vi "Merge Limelight Data.vi"() -> ()   [LabVIEW 2025]
uses:
  <vilib>/Rock Robotics/WPI/DriverStation/WPI_DriverStationRobotMode2.ctl
  <vilib>/Rock Robotics/Network Tables/NT Read Numeric Array.vi
  <vilib>/Rock Robotics/Network Tables/NT Read Number.vi
  <vilib>/Rock Robotics/Network Tables/NT Write Numeric Array.vi
  Framework/Robot Global Data.vi
  <vilib>/Rock Robotics/Network Tables/NT Write String.vi
panel:
  out "What Camera are we seeing out of?":i32
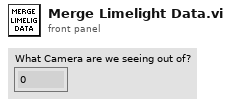
[diagram p1: front panel]
types:
  T1 = typedef "WPI_DriverStationRobotMode2.ctl" = enum16{"Autonomous Disabled", "Autonomous Enabled", "Teleop Disabled", "Teleop Enabled", "Disconnected", "Finish", "Test Disabled", "Test Enabled", "Emergency Stopped"}
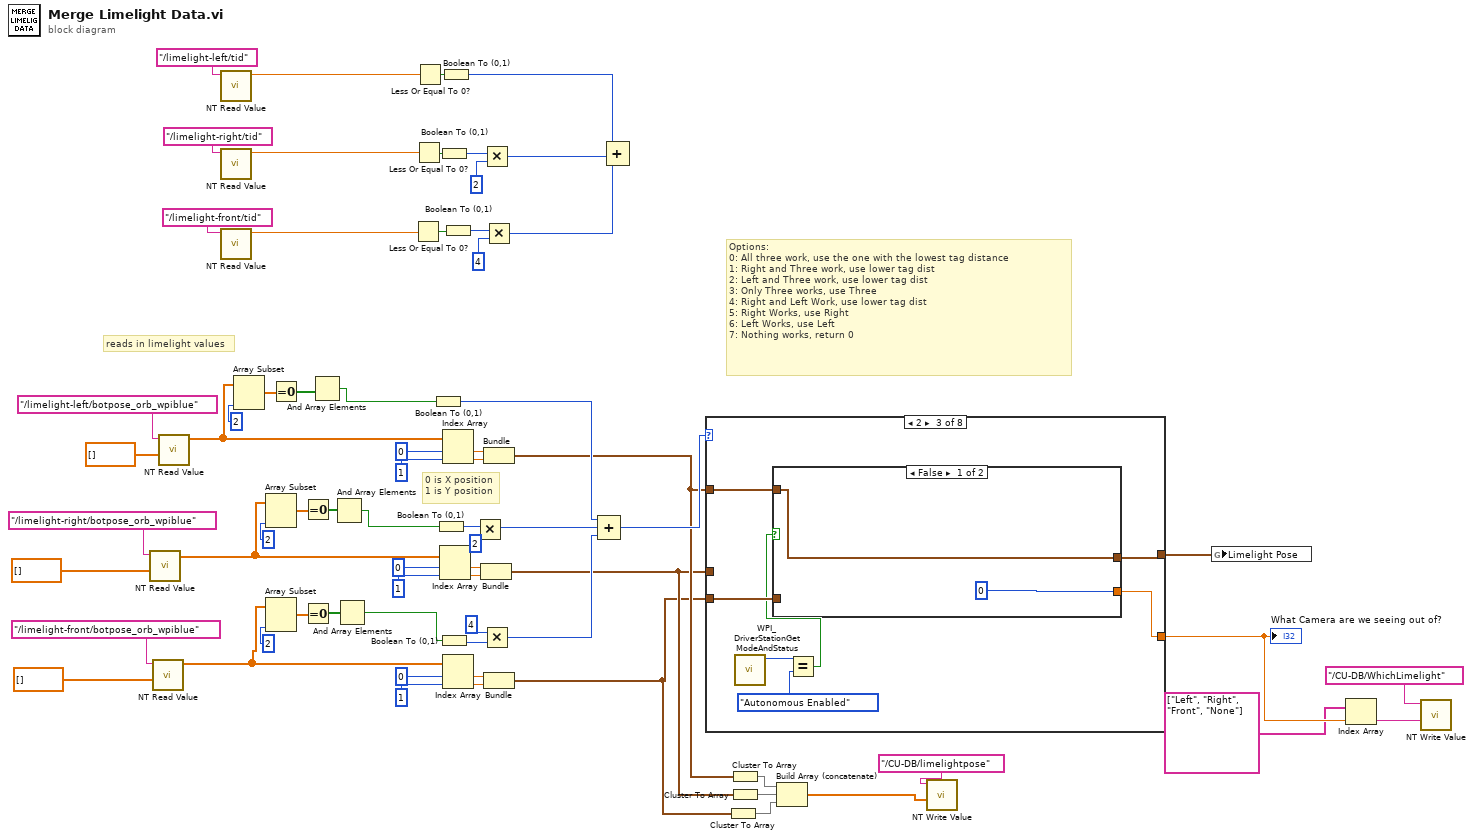
[diagram p0: block diagram]
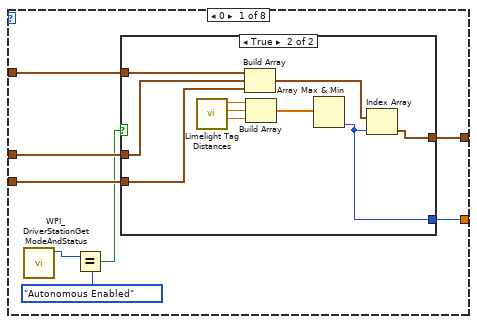
[diagram p2: hidden frame]
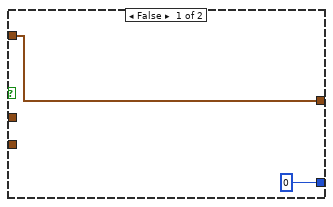
[diagram p3: hidden frame]
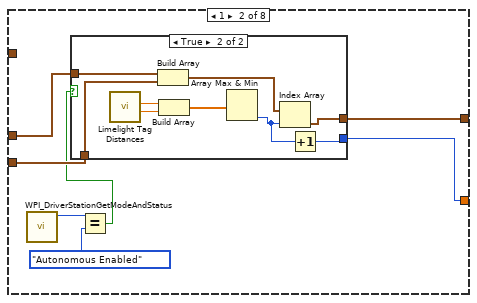
[diagram p4: hidden frame]
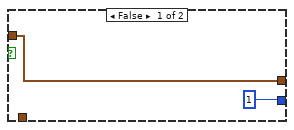
[diagram p5: hidden frame]
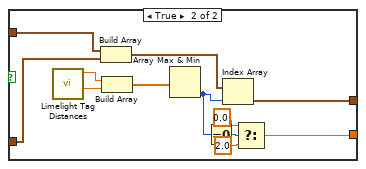
[diagram p6: hidden frame]
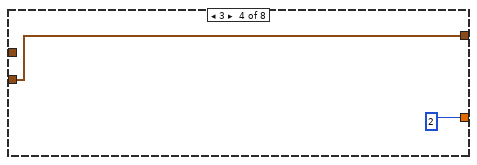
[diagram p7: hidden frame]
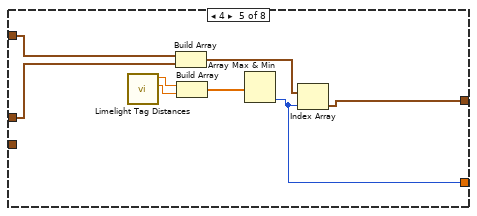
[diagram p8: hidden frame]
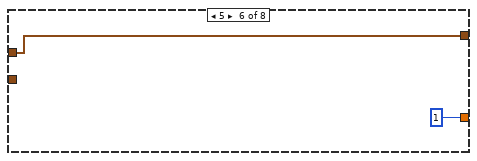
[diagram p9: hidden frame]
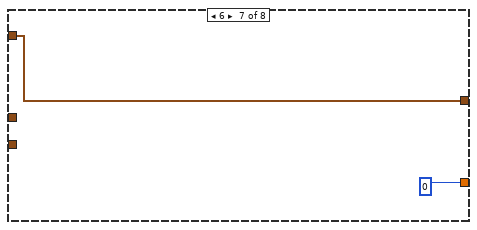
[diagram p10: hidden frame]
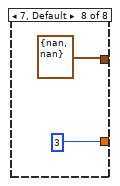
[diagram p11: hidden frame]
diagram:
  # "Options:\n0: All three work, use the one with the lowest tag distance\n1: Right and Three work, use lower tag dist\n2: Left and Three work, use lower tag dist\n3: Only Three works, use Three\n4: Right and Left Work, use lower tag dist\n5: Right Works, use Right\n6: Left Works, use Left\n7: Nothing works, return 0"
  # "reads in limelight values"
  # "0 is X position\n1 is Y position"
  n1 = call-poly <vilib>:"NT Read Value.vi"("default value"=dbl[] [], "name"="/limelight-right/botpose_orb_wpiblue") -> ("value"=w22:dbl[])  [unwired: 7 in, 2 out]
  n2 = call-poly <vilib>:"NT Read Value.vi"("default value"=dbl[] [], "name"="/limelight-front/botpose_orb_wpiblue") -> ("value"=w19:dbl[])  [unwired: 7 in, 2 out]
  n3 = call-poly <vilib>:"NT Read Value.vi"("default value"=dbl[] [], "name"="/limelight-left/botpose_orb_wpiblue") -> ("value"=w27:dbl[])  [unwired: 7 in, 2 out]
  n4 = call-poly <vilib>:"NT Read Value.vi"("name"="/limelight-left/tid") -> ("value"=w45:dbl)  [unwired: 8 in, 2 out]
  n5 = call-poly <vilib>:"NT Read Value.vi"("name"="/limelight-right/tid") -> ("value"=w44:dbl)  [unwired: 8 in, 2 out]
  n6 = call-poly <vilib>:"NT Read Value.vi"("name"="/limelight-front/tid") -> ("value"=w43:dbl)  [unwired: 8 in, 2 out]
  n7 = Array Subset(array=w27, length=2) -> (w25:dbl[])  [unwired: 1 in]
  n8 = Array Subset(array=w22, length=2) -> (w23:dbl[])  [unwired: 1 in]
  n9 = Array Subset(array=w19, length=2) -> (w20:dbl[])  [unwired: 1 in]
  n10 = Equal To 0?(x=w25) -> (x = 0?=w13:bool[])
  n11 = Equal To 0?(x=w23) -> (x = 0?=w15:bool[])
  n12 = Equal To 0?(x=w20) -> (x = 0?=w17:bool[])
  n13 = And Array Elements(Boolean array=w13) -> (logical AND=w12:bool)
  n14 = And Array Elements(Boolean array=w15) -> (logical AND=w14:bool)
  n15 = And Array Elements(Boolean array=w17) -> (logical AND=w16:bool)
  n16 = Less Or Equal To 0?(x=w43) -> (x <= 0?=w42:bool)
  n17 = Less Or Equal To 0?(x=w44) -> (x <= 0?=w41:bool)
  n18 = Less Or Equal To 0?(x=w45) -> (x <= 0?=w40:bool)
  n19 = Boolean To (0,1)(Boolean=w12) -> (0, 1=w30:i16)
  n20 = Boolean To (0,1)(Boolean=w14) -> (0, 1=w50:i16)
  n21 = Boolean To (0,1)(Boolean=w41) -> (0, 1=w37:i16)
  n22 = Boolean To (0,1)(Boolean=w16) -> (0, 1=w52:i16)
  n23 = Index Array(array=w22, index #1=0 ("index"), index #2=1 ("index")) -> (element #1=w64:dbl, element #2=w65:dbl)
  n24 = Boolean To (0,1)(Boolean=w40) -> (0, 1=w39:i16)
  n25 = Boolean To (0,1)(Boolean=w42) -> (0, 1=w34:i16)
  n26 = Index Array(array=w27, index #1=0 ("index"), index #2=1 ("index")) -> (element #1=w69:dbl, element #2=w70:dbl)
  n27 = Index Array(array=w19, index #1=0 ("index"), index #2=1 ("index")) -> (element #1=w57:dbl, element #2=w56:dbl)
  n28 = Multiply(x=w50, y=i16 2) -> (x*y=w29:i16)
  n29 = Bundle("Numeric"=w64, "Numeric"=w65) -> (w10:cluster{"Numeric":dbl, "Numeric":dbl})  [unwired: 1 in]
  n30 = Multiply(x=w37, y=i16 2) -> (x*y=w32:i16)
  n31 = Multiply(x=i16 4, y=w52) -> (x*y=w28:i16)
  n32 = Multiply(x=w34, y=i16 4) -> (x*y=w33:i16)
  n33 = Bundle("Numeric"=w69, "Numeric"=w70) -> (w11:cluster{"Numeric":dbl, "Numeric":dbl})  [unwired: 1 in]
  n34 = Bundle("Numeric"=w57, "Numeric"=w56) -> (w9:cluster{"Numeric":dbl, "Numeric":dbl})  [unwired: 1 in]
  n35 = Compound Arithmetic op=ADD(w30, w29, w28) -> (w18:i16)
  n36 = Compound Arithmetic op=ADD(w39, w32, w33) -> ()  [unwired: 1 out]
  n37 = case shown="2" w18 {
    tunnel: w11 -> [w78 _ w115 _ w137 _ w143 _]
    tunnel: w10 -> [w77 w97 _ _ w136 w141 _ _]
    tunnel: w9 -> [w76 w96 w114 w131 _ _ _ _]
    tunnel: [w75 w95 w113 w131 w133 w141 w143 cluster{"Numeric":dbl, "Numeric":dbl} {"Numeric"=nan, "Numeric"=nan}] -> w31
    tunnel: [w71 w91 w109 2 w132 1 0 3] -> w4
    frame 0 {
      n38 = call <vilib>:"WPI_DriverStationGetModeAndStatus.vi"() -> ("Robot Mode"=w74:T1)  [unwired: 10 in, 1 out]
      n39 = Equal?(x=w74, y=WPI_DriverStationRobotMode2."Autonomous Enabled") -> (x = y?=w72:bool)
      n40 = case shown="True" w72 {
        tunnel: w78 -> [w80 w86]
        tunnel: w77 -> [_ w85]
        tunnel: w76 -> [_ w84]
        tunnel: [w80 w82] -> w75
        tunnel: [0 w81] -> w71
        frame False {
        }
        frame True {
          n41 = call "Limelight Tag Distances.vi"() -> ("Front"=w89:dbl, "Right"=w90:dbl, "Left"=w87:dbl)  [unwired: 9 in]
          n42 = Build Array(w86, w85, w84) -> (w83:cluster{"Numeric":dbl, "Numeric":dbl}[])
          n43 = Build Array(w87, w90, w89) -> (w88:dbl[])
          n44 = Array Max & Min(array=w88) -> (min index (indices)=w81:i32)  [unwired: 3 out]
          n45 = Index Array(array=w83, index=w81) -> (element=w82:cluster{"Numeric":dbl, "Numeric":dbl})
        }
      }
    }
    frame 1 {
      n46 = call <vilib>:"WPI_DriverStationGetModeAndStatus.vi"() -> ("Robot Mode"=w94:T1)  [unwired: 10 in, 1 out]
      n47 = Equal?(x=w94, y=WPI_DriverStationRobotMode2."Autonomous Enabled") -> (x = y?=w92:bool)
      n48 = case shown="True" w92 {
        tunnel: w97 -> [w99 w104]
        tunnel: w96 -> [_ w103]
        tunnel: [w99 w102] -> w95
        tunnel: [1 w101] -> w91
        frame False {
        }
        frame True {
          n49 = call "Limelight Tag Distances.vi"() -> ("Front"=w107:dbl, "Right"=w108:dbl)  [unwired: 9 in, 1 out]
          n50 = Build Array(w104, w103) -> (w105:cluster{"Numeric":dbl, "Numeric":dbl}[])
          n51 = Build Array(w108, w107) -> (w106:dbl[])
          n52 = Array Max & Min(array=w106) -> (min index (indices)=w100:i32)  [unwired: 3 out]
          n53 = Index Array(array=w105, index=w100) -> (element=w102:cluster{"Numeric":dbl, "Numeric":dbl})
          n54 = Increment(x=w100) -> (x+1=w101:i32)
        }
      }
    }
    frame 2 {
      n55 = call <vilib>:"WPI_DriverStationGetModeAndStatus.vi"() -> ("Robot Mode"=w112:T1)  [unwired: 10 in, 1 out]
      n56 = Equal?(x=w112, y=WPI_DriverStationRobotMode2."Autonomous Enabled") -> (x = y?=w110:bool)
      n57 = case shown="False" w110 {
        tunnel: w115 -> [w117 w125]
        tunnel: w114 -> [_ w124]
        tunnel: [w117 w123] -> w113
        tunnel: [0 w122] -> w109
        frame False {
        }
        frame True {
          n58 = call "Limelight Tag Distances.vi"() -> ("Front"=w129:dbl, "Left"=w126:dbl)  [unwired: 9 in, 1 out]
          n59 = Build Array(w125, w124) -> (w127:cluster{"Numeric":dbl, "Numeric":dbl}[])
          n60 = Build Array(w126, w129) -> (w128:dbl[])
          n61 = Array Max & Min(array=w128) -> (min index (indices)=w120:i32)  [unwired: 3 out]
          n62 = Equal To 0?(x=w120) -> (x = 0?=w121:bool)
          n63 = Index Array(array=w127, index=w120) -> (element=w123:cluster{"Numeric":dbl, "Numeric":dbl})
          n64 = Select(t=0.0, s=w121, f=2.0) -> (s? t:f=w122:dbl)
        }
      }
    }
    frame 3 {
    }
    frame 4 {
      n65 = call "Limelight Tag Distances.vi"() -> ("Right"=w134:dbl, "Left"=w135:dbl)  [unwired: 9 in, 1 out]
      n66 = Build Array(w137, w136) -> (w138:cluster{"Numeric":dbl, "Numeric":dbl}[])
      n67 = Build Array(w135, w134) -> (w139:dbl[])
      n68 = Array Max & Min(array=w139) -> (min index (indices)=w132:i32)  [unwired: 3 out]
      n69 = Index Array(array=w138, index=w132) -> (element=w133:cluster{"Numeric":dbl, "Numeric":dbl})
    }
    frame 5 {
    }
    frame 6 {
    }
    frame 7, Default {
    }
  }
  "What Camera are we seeing out of?" <- w4
  n70 = Cluster To Array(cluster=w9) -> (array=w6:dbl[])
  n71 = Cluster To Array(cluster=w11) -> (array=w8:dbl[])
  n72 = Cluster To Array(cluster=w10) -> (array=w7:dbl[])
  n73 = Build Array (concatenate)(w8, w7, w6) -> (w5:dbl[])
  n74 = call-poly <vilib>:"NT Write Value.vi"("value"=w5, "name"="/CU-DB/limelightpose") -> ()  [unwired: 9 in, 1 out]
  n75 = global write "Robot Global Data.vi" "Limelight Pose"(w31) -> ()
  n76 = Index Array(array=string[] ["Left", "Right", "Front", "None"], index=w4) -> (element=w2:string)
  n77 = call-poly <vilib>:"NT Write Value.vi"("value"=w2, "name"="/CU-DB/WhichLimelight") -> ()  [unwired: 9 in, 1 out]
